vi "Highlight State Call.vi"(8 "error in (no error)":errorcluster, 10 "State Call":T1, 11 "JKI SM in":refnum<class "JKI SM.lvclass">) -> (0 "error out":errorcluster, 3 "JKI SM out":refnum<class "JKI SM.lvclass">)   [LabVIEW 2020]
uses:
  JKI State Machine API/source/JKI SM/JKI SM.lvclass
  JKI State Machine API/source/Support/State Call Cluster.ctl
  7cc11248-e9f2-4ae1-800a-eb99d6b5ead2.vi
  9de462b7-3281-44a3-b461-53614e7f228c.vi
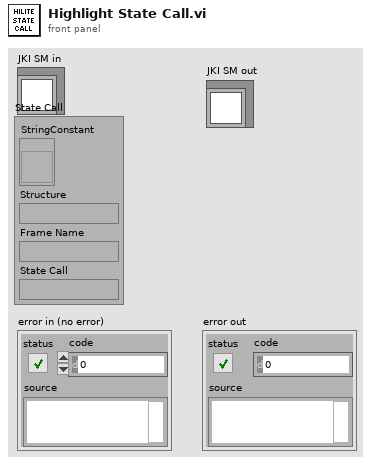
[diagram p1: front panel]
types:
  T1 = typedef "State Call Cluster.ctl" = cluster{"StringConstant":refnum<vi>, "Structure":string, "Frame Name":string, "State Call":string}
  T2 = typedef "LVFontTypeDef.ctl" = cluster{"Font Name":string, "Size":u16, "Bold":bool, "Italic":bool, "Underline":bool, "Strikeout":bool, "Color":u32}
  T3 = typedef "LVTextColorsTypeDef.ctl" = cluster{"Text Color":u32, "Background Color":u32}
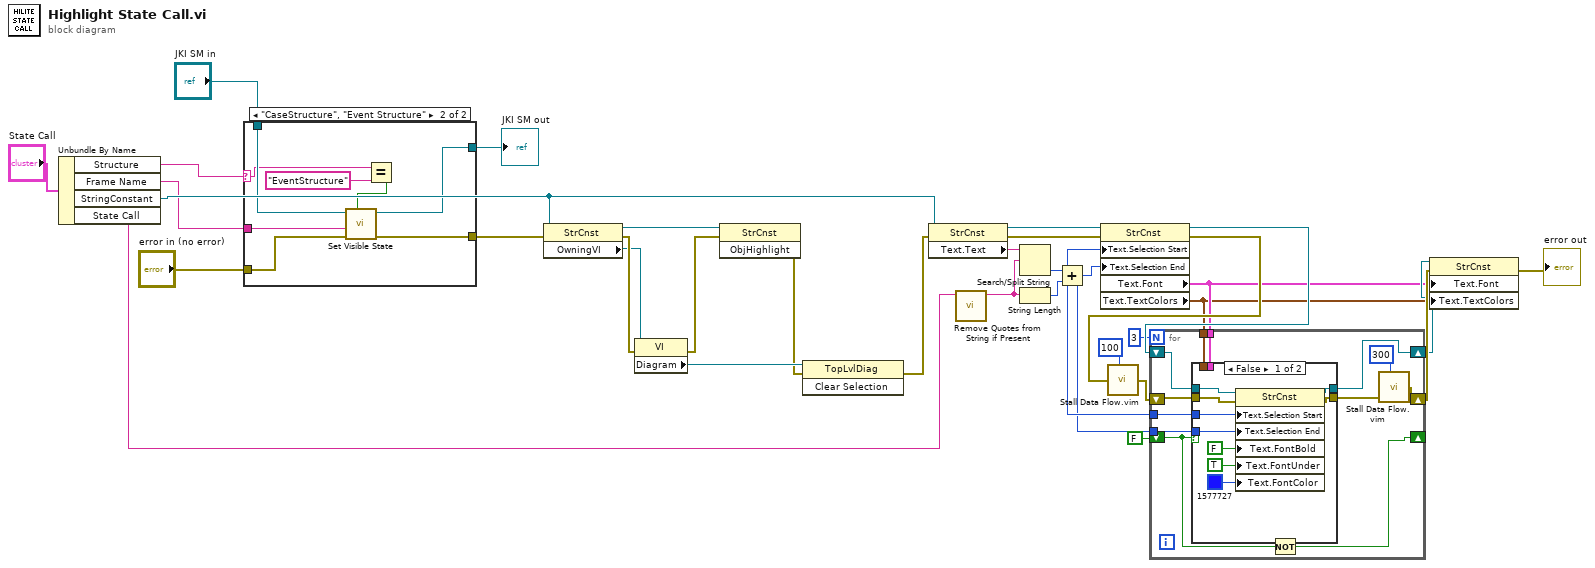
[diagram p0: block diagram]
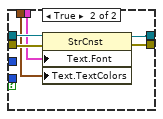
[diagram p3: hidden frame]
diagram:
  n1 = Unbundle By Name("State Call") -> ("Structure"=w8:string, "Frame Name"=w9:string, "StringConstant"=w13:refnum<vi>, "State Call"=w7:string)
  n2 = case shown="\"CaseStructure\", \"Event Structure\"" w8 {
    selector: w8 -> [_ w38]
    tunnel: [w35 w44] -> w34
    tunnel: "error in (no error)" -> [w35 w43]
    tunnel: "JKI SM in" -> [w36 w42]
    tunnel: [w36 w41] -> w30
    tunnel: w9 -> [_ w40]
    frame Default {
      # "No Fram"
    }
    frame "CaseStructure", "Event Structure" {
      n3 = Equal?(x=w38, y="EventStructure") -> (x = y?=w37:bool)
      n4 = call "Set Visible State.vi"("Event Structure (F: Case Structure)"=w37, "error in (no error)"=w43, "State Name"=w40, "JKI SM in"=w42) -> ("error out"=w44:errorcluster, "JKI SM out"=w41:refnum<class "JKI SM.lvclass">)  [unwired: 6 in]
    }
  }
  "JKI SM out" <- w30
  n5 = property class="StrCnst"(reference=w13, error in=w34) -> (reference out=w1:refnum<vi>, error out=w4:errorcluster, "OwningVI"=w3:refnum<vi>)
  n6 = property class="VI"(reference=w3, error in=w4) -> (error out=w5:errorcluster, "Diagram"=w6:refnum<vi>)  [unwired: 1 out]
  n7 = invoke class="StrCnst" method="ObjHighlight"(reference=w1, error in=w5) -> (error out=w2:errorcluster)  [unwired: 1 in, 2 out]
  n8 = invoke class="TopLvlDiag" method="Clear Selection"(reference=w6, error in=w2) -> (error out=w26:errorcluster)  [unwired: 1 in, 2 out]
  n9 = property class="StrCnst"(reference=w13, error in=w26) -> (reference out=w28:refnum<vi>, error out=w25:errorcluster, "Text.Text"=w29:string)
  n10 = call "Remove Quotes from String if Present.vi"("String"=w7) -> ("String with Quotes Removed"=w24:string)  [unwired: 10 in]
  n11 = Search/Split String(string=w29, search string/char (-)=w24) -> (offset of match=w11:i32)  [unwired: 1 in, 2 out]
  n12 = String Length(string=w24) -> (length=w27:i32)
  n13 = Add(x=w11, y=w27) -> (x+y=w10:i32)
  n14 = property class="StrCnst"(reference=w28, error in=w25, "Text.Selection Start"=w11, "Text.Selection End"=w10) -> (reference out=w23:refnum<vi>, error out=w17:errorcluster, "Text.Font"=w14:T2, "Text.TextColors"=w12:T3)
  n15 = call "Stall Data Flow.vim"("value in"=w17, "milliseconds to wait"=u32 100) -> ("value out"=w18:errorcluster)  [unwired: 1 out]
  n16 = for {
    N: 3 -> [_]
    shift-right: [w53] -> w22
    shift-left: w18 -> [w51]
    shift-right: [w52] -> w20
    shift-left: w23 -> [w56]
    shift-right: [w49] -> _
    shift-left: FALSE -> [w50]
    tunnel: w14 -> [w48]
    tunnel: w12 -> [w47]
    tunnel: w11 -> [w46]
    tunnel: w10 -> [w45]
    n17 = case shown="False" w50 {
      tunnel: w56 -> [w65 w71]
      tunnel: [w64 w69] -> w55
      tunnel: [w63 w70] -> w52
      tunnel: w51 -> [w60 w68]
      tunnel: w48 -> [_ w67]
      tunnel: w47 -> [_ w66]
      tunnel: w46 -> [w58 _]
      tunnel: w45 -> [w57 _]
      frame False {
        n18 = property class="StrCnst"(reference=w65, error in=w60, "Text.Selection Start"=w58, "Text.Selection End"=w57, "Text.FontBold"=FALSE ("Text.Font:Bold"), "Text.FontUnder"=TRUE ("Text.Font:Bold"), "Text.FontColor"=u32 1577727) -> (reference out=w63:refnum<vi>, error out=w64:errorcluster)
      }
      frame True {
        n19 = property class="StrCnst"(reference=w71, error in=w68, "Text.Font"=w67, "Text.TextColors"=w66) -> (reference out=w70:refnum<vi>, error out=w69:errorcluster)
      }
    }
    n20 = Not(x=w50) -> (.not. x?=w49:bool)
    n21 = call "Stall Data Flow.vim"("value in"=w55, "milliseconds to wait"=u32 300) -> ("value out"=w53:errorcluster)  [unwired: 1 out]
  }
  n22 = property class="StrCnst"(reference=w20, error in=w22, "Text.Font"=w14, "Text.TextColors"=w12) -> (error out=→"error out":errorcluster)  [unwired: 1 out]
